vi "set_table.vi"(8 "error in (no error)":errorcluster, 9 "Table":refnum<class "Table.lvclass">, 10 "table_name":string, 11 "Doc in":refnum<class "Doc.lvclass">) -> (0 "error out":errorcluster, 3 "Doc out":refnum<class "Doc.lvclass">)   [LabVIEW 2020, in "toml_edit.lvlib" / "Doc.lvclass"]
uses:
  Doc.lvclass
  Table/Table.lvclass
  Doc.lvclass/Doc.ctl
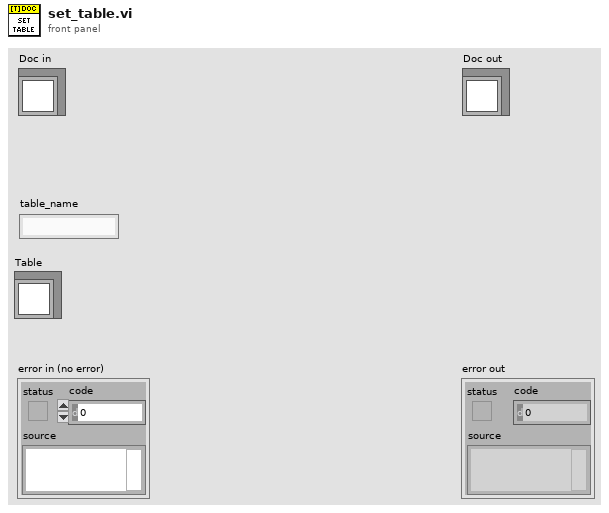
[diagram p1: front panel]
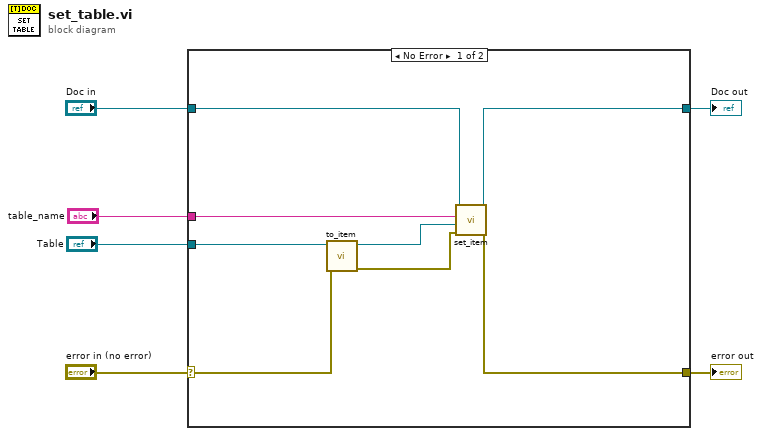
[diagram p0: block diagram]
diagram:
  n1 = case shown="No Error" "error in (no error)" {
    selector: "error in (no error)" -> [w12 w16]
    tunnel: [w7 w16] -> w5
    tunnel: [w11 w15] -> w3
    tunnel: "Doc in" -> [w10 w15]
    tunnel: "table_name" -> [w13 _]
    tunnel: "Table" -> [w9 _]
    frame No Error {
      n2 = call "to_item.vi"("error in (no error)"=w12, "Table in"=w9) -> ("error out"=w14:errorcluster, "Item out"=w8:refnum<class "Item.lvclass">)  [unwired: 8 in]
      n3 = call "set_item.vi"("error in (no error)"=w14, "Item"=w8, "item_name"=w13, "Doc in"=w10) -> ("error out"=w7:errorcluster, "Doc out"=w11:refnum<class "Doc.lvclass">)  [unwired: 6 in]
    }
    frame Error {
    }
  }
  "error out" <- w5
  "Doc out" <- w3
